vi "MQTT Subscriptions - Handle Unsuback.vi"(0 "MQTT ref in":T1, 5 "Packet ID":u16, 7 "Reason Codes":u8[](array[numeric]), 9 "Reason String":string) -> (4 "MQTT ref out":T1)   [LabVIEW 2019, in "KoRE-MQTT.lvlib"]
doc: "Copyright (c) 2025 KoRElibs.com\nSPDX-License-Identifier: EUPL-1.2\n\nThis VI is licensed under the European Union Public License (EUPL) Version 1.2. You may use this VI unmodified in proprietary works. If you distribute a modified version of this file, the modified file must be released under the EUPL-1.2. Full license: https://joinup.ec.europa.eu/asset/eupl/eupl/1.2/"
uses:
  KoRE-MQTT.lvlib
  Public/TypeDefs/MQTT Client Session.ctl
  TypeDefs/MQTT Client Session - Data Value Reference.ctl
  Public/TypeDefs/MQTT Client Session - Data.ctl
  Public/TypeDefs/MQTT Property - Will.ctl
  Public/TypeDefs/MQTT Property - CONNECT.ctl
  TypeDefs/MQTT Subscription - Info.ctl
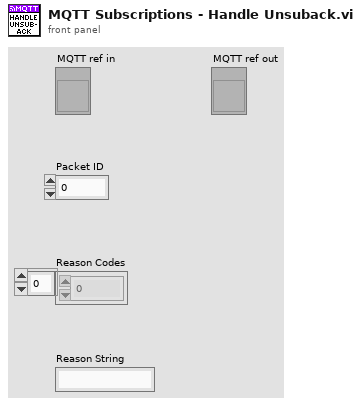
[diagram p1: front panel]
types:
  T1 = typedef "KoRE-MQTT.lvlib/MQTT Client Session.ctl" = refnum<vi>
  T2 = typedef "KoRE-MQTT.lvlib/MQTT Client Session - Data Value Reference.ctl" = refnum<data-value>
  T3 = typedef "KoRE-MQTT.lvlib/MQTT Client Session - Data.ctl" = cluster{"TCP ref":refnum<k5>, "Next Packet Id":u16, "Version":u8, "Host":string, "Port":u16, "Ping Delta":u32, "Username":string, "Password":string, "Will QoS":u8, "Will Retain":bool, "Will Topic":string, "Will Payload":string, "TCP Timeout":i32, "Semaphore":T4, "In-Flight Messages":variant, "Close":bool, "Last Send":u32, "Keep Alive":u16, "Last Ping RTT":u32, "Last Ping":u32, "Will Properties":T5[], "Session Expiry Interval":u32, "Maximum QoS":u8, "Retain Available":bool, "Server Maximum Packet Size":u32, "Client Identifier":string, "Server Topic Alias Maximum":u16, "Wildcard Subscription Available":bool, "Subscription Identifier Available":bool, "Shared Subscription Available":bool, "Connect Properties":T6[], "Client Maximum Packet Size":u32, "Client Topic Alias Maximum":u16, "Server Receive Maximum":u16, "Client Receive Maximum":u16, "TLS cfg":refnum<k36>, "Subscriptions":T7[]}
  T4 = typedef "Semaphore RefNum" = refnum<k1>
  T5 = typedef "KoRE-MQTT.lvlib/MQTT Property - Will.ctl" = cluster{"Property":u8, "Value":string}
  T6 = typedef "KoRE-MQTT.lvlib/MQTT Property - CONNECT.ctl" = cluster{"Property":u8, "Value":string}
  T7 = typedef "KoRE-MQTT.lvlib/MQTT Subscription - Info.ctl" = cluster{"Packet Id":u16, "Index":u16, "Identifier":u32, "QoS":u8, "Topic Filter":string, "Reason Code":u8, "Reason String":string, "Granted":bool}
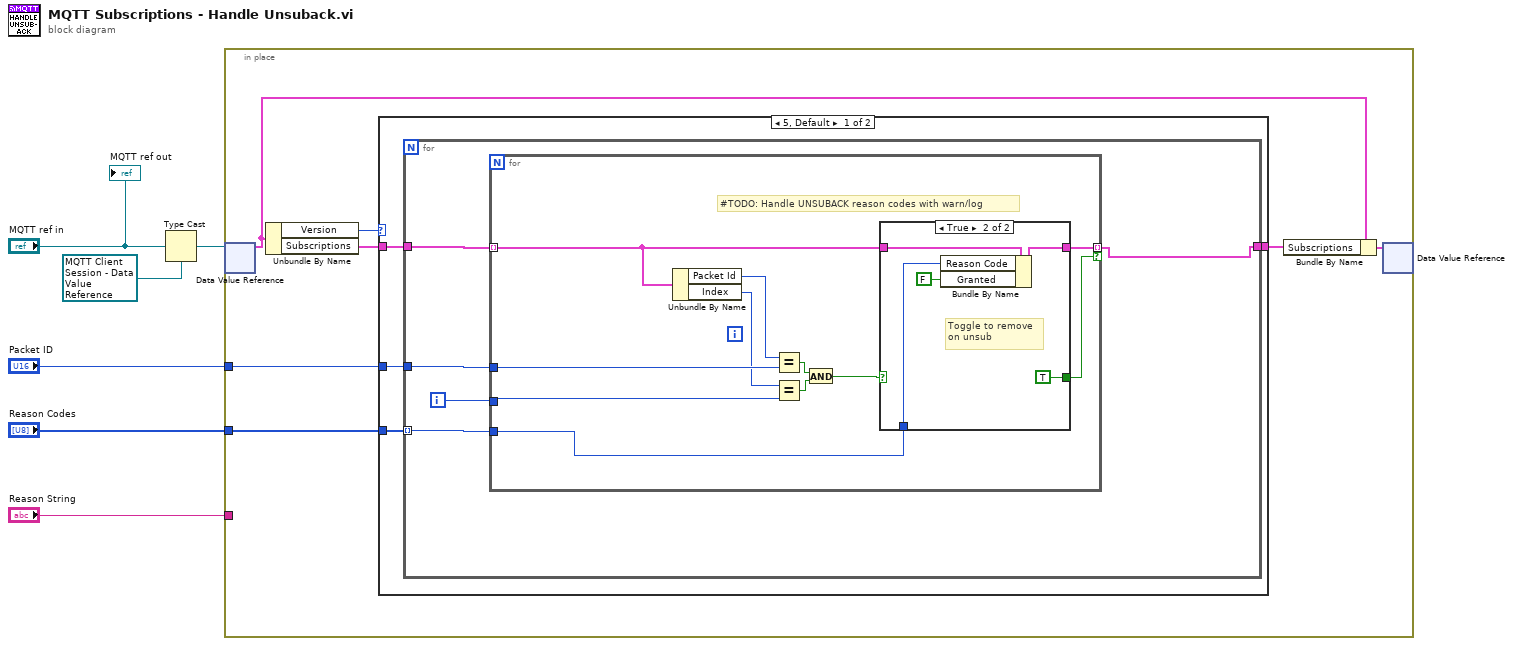
[diagram p0: block diagram]
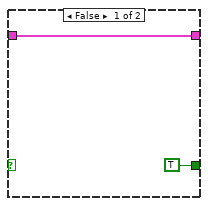
[diagram p2: hidden frame]
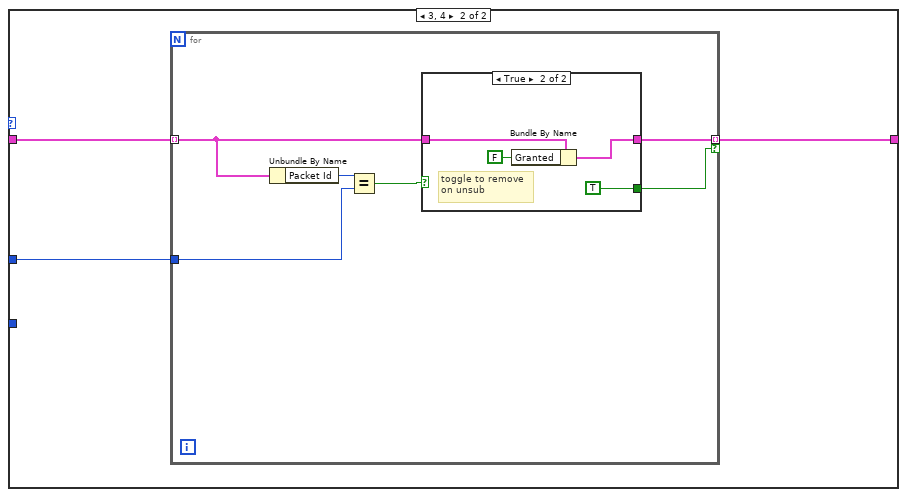
[diagram p3: hidden frame]
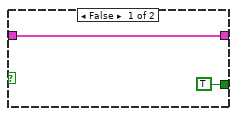
[diagram p4: hidden frame]
diagram:
  n1 = Type Cast(type=T2 refnum ("data value reference"), x="MQTT ref in") -> (*(type *) &x=w3:T2)
  n2 = in-place {
    in-place-border: "Packet ID" -> [w8]
    in-place-border: "Reason Codes" -> [w7]
    in-place-border: "Reason String" -> [_]
    n3 = in-place-dvr #1(w3) -> (w12:T3)  [unwired: 1 out]
    n4 = Unbundle By Name(w12) -> ("Version"=w11:u8, "Subscriptions"=w10:T7[])
    n5 = case shown="5, Default" w11 {
      tunnel: w10 -> [w16 w43]
      tunnel: [w15 w42] -> w9
      tunnel: w8 -> [w14 w41]
      tunnel: w7 -> [w17 _]
      frame 5, Default {
        n6 = for {
          tunnel: w17 -> [w18] mode=indexing
          tunnel: w16 -> [w22]
          tunnel: [w21] -> w15
          tunnel: w14 -> [w20]
          i -> [w19]
          n7 = for {
            tunnel: w22 -> [w33] mode=indexing
            tunnel: [w32] -> w21 mode=indexing if=w24
            tunnel: w20 -> [w31]
            tunnel: w19 -> [w30]
            tunnel: w18 -> [w29]
            # "#TODO: Handle UNSUBACK reason codes with warn/log"
            n8 = Unbundle By Name(w33) -> ("Packet Id"=w28:u16, "Index"=w27:u16)
            n9 = Equal?(x=w28, y=w31) -> (x = y?=w25:bool)
            n10 = Equal?(x=w27, y=w30) -> (x = y?=w26:bool)
            n11 = And(x=w25, y=w26) -> (x .and. y?=w23:bool)
            n12 = case shown="True" w23 {
              tunnel: w33 -> [w34 w40]
              tunnel: [w34 w39] -> w32
              tunnel: w29 -> [_ w38]
              tunnel: [TRUE TRUE] -> w24
              frame False {
              }
              frame True {
                # "Toggle to remove\non unsub"
                n13 = Bundle By Name(cluster=w40, "Reason Code"=w38, "Granted"=FALSE) -> (w39:T7)
              }
            }
          }
        }
      }
      frame 3, 4 {
        n14 = for {
          tunnel: w43 -> [w47] mode=indexing
          tunnel: [w46] -> w42 mode=indexing if=w44
          tunnel: w41 -> [w48]
          n15 = Unbundle By Name(w47) -> ("Packet Id"=w49:u16)
          n16 = Equal?(x=w49, y=w48) -> (x = y?=w45:bool)
          n17 = case shown="True" w45 {
            tunnel: w47 -> [w51 w55]
            tunnel: [w51 w54] -> w46
            tunnel: [TRUE TRUE] -> w44
            frame False {
            }
            frame True {
              # "toggle to remove\non unsub"
              n18 = Bundle By Name(cluster=w55, "Granted"=FALSE) -> (w54:T7)
            }
          }
        }
      }
    }
    n19 = Bundle By Name(cluster=w12, "Subscriptions"=w9) -> (w13:T3)
    n20 = in-place-dvr #1(w13) -> ()  [unwired: 2 out]
  }
  "MQTT ref out" <- "MQTT ref in"
